vi "fake tool array shapes.vi"(6 "cluster with array":cluster{"values":dbl[]}, 7 "clusterarray":cluster{"x":dbl, "name":string}[](array[cluster]), 8 "enumarray":enum16{"red", "green", "blue"}[](array[ring]), 9 "patharray":path[](array[path]), 10 "timestamparray":timestamp[](array[timestamp]), 11 "array3d":dbl[][][](array[numeric])) -> (3 "result string":string)   [LabVIEW 2020, in "MCP Server tests.lvlib"]
doc: "Fake tool to test that tools/list describes every array input with items, for array shapes beyond 1D arrays of plain numbers, strings and Booleans: a 3D array, arrays of timestamps, paths, enums and clusters, and a cluster that contains an array. It returns its inputs flattened to XML."
uses:
  MCP Server tests.lvlib
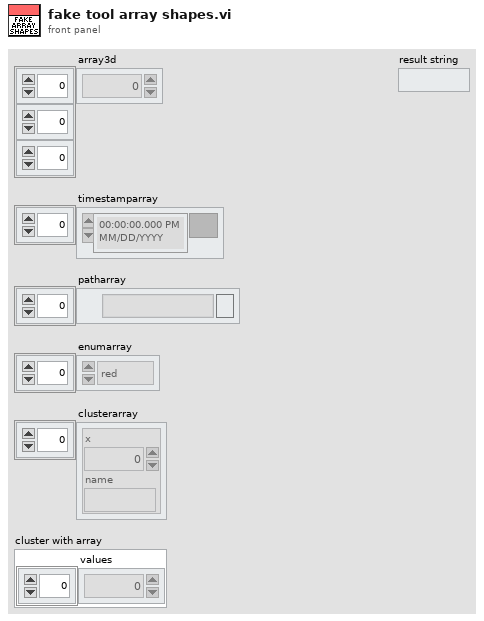
[diagram p1: front panel]
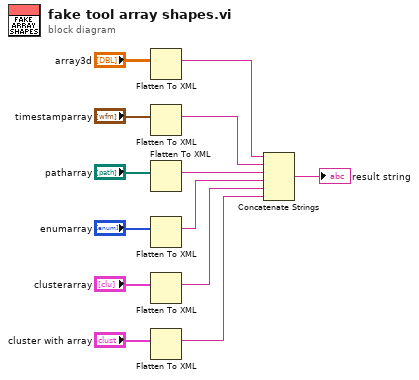
[diagram p0: block diagram]
diagram:
  n1 = Flatten To XML(6:"array3d") -> (2:w7:string)
  n2 = Flatten To XML(6:"timestamparray") -> (2:w6:string)
  n3 = Flatten To XML(6:"patharray") -> (2:w5:string)
  n4 = Flatten To XML(6:"enumarray") -> (2:w4:string)
  n5 = Flatten To XML(6:"clusterarray") -> (2:w3:string)
  n6 = Flatten To XML(6:"cluster with array") -> (2:w2:string)
  n7 = Concatenate Strings(w7, w6, w5, w4, w3, w2) -> (→"result string":string)
